vi "Server.vi"() -> ()   [LabVIEW 2020]
uses:
  source/PV Data/NT Scalar (Numeric)/NT Scalar (Numeric).lvclass
  C:/Users/eyw68381/source/repos/pvaccess-labview/labview/source/PV Data/NT Scalar/NT Scalar.lvclass
  C:/Users/eyw68381/source/repos/pvaccess-labview/labview/source/PV Data/NT Base/NT Base.lvclass
  C:/Users/eyw68381/source/repos/pvaccess-labview/labview/source/PV Data/Base/Base.lvclass
  C:/Users/eyw68381/source/repos/pvaccess-labview/labview/source/PV Data/Has Alarm Limits/Has Alarm Limits.lvclass
  C:/Users/eyw68381/source/repos/pvaccess-labview/labview/source/PV Data/Base Interface/Base Interface.lvclass
  C:/Users/eyw68381/source/repos/pvaccess-labview/labview/source/PV Data/Has Control Limits/Has Control Limits.lvclass
  C:/Users/eyw68381/source/repos/pvaccess-labview/labview/source/PV Data/Is Stringifiable/Is Stringifiable.lvclass
  C:/Users/eyw68381/source/repos/pvaccess-labview/labview/source/PV Data/Is Probeable/Is Probeable.lvclass
  C:/Users/eyw68381/source/repos/pvaccess-labview/labview/source/PV Data/Has Alarm/Has Alarm.lvclass
  C:/Users/eyw68381/source/repos/pvaccess-labview/labview/source/PV Data/Has Time Stamp/Has Time Stamp.lvclass
  C:/Users/eyw68381/source/repos/pvaccess-labview/labview/source/PV Data/NT Scalar (Numeric)/NT Scalar (Numeric).lvclass
  source/Server/Server/Server.lvclass
  source/PV Data/Value Fields.ctl
  source/PV Data/PV Data.lvlib
  source/PV Data/Alarm Severity.ctl
  source/PV Data/Display Form.ctl
  source/Server/Server/Post - DBL.vi
  source/Server/Server/Fetch - DBL.vi
  source/Server/Server/Add PV - Any Class.vi
  source/PV Data/NT Scalar (Numeric)/Create - DBL.vi
panel:
  in  "PV name":string="DEV:FLOAT64"
  out "timestamp":timestamp
  in  "Value":dbl min=0.0 max=10.0 step=0.5 format="%.3f"
  in  "Increment":bool
  in  "stop":bool
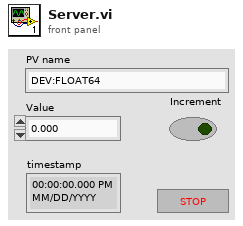
[diagram p1: front panel]
types:
  T1 = typedef "PV Access.lvlib/PV Data.lvlib/Value Fields.ctl" = cluster{"Display":bool, "Control":bool, "Alarm Limits":bool}
  T2 = typedef "PV Access.lvlib/PV Data.lvlib/Alarm Severity.ctl" = enum32{"no", "minor", "major", "record", "invalid", "undefined"}
  T3 = typedef "PV Access.lvlib/PV Data.lvlib/Display Form.ctl" = enum16{"Default", "String", "Binary", "Decimal", "Hex", "Exponential", "Engineering"}
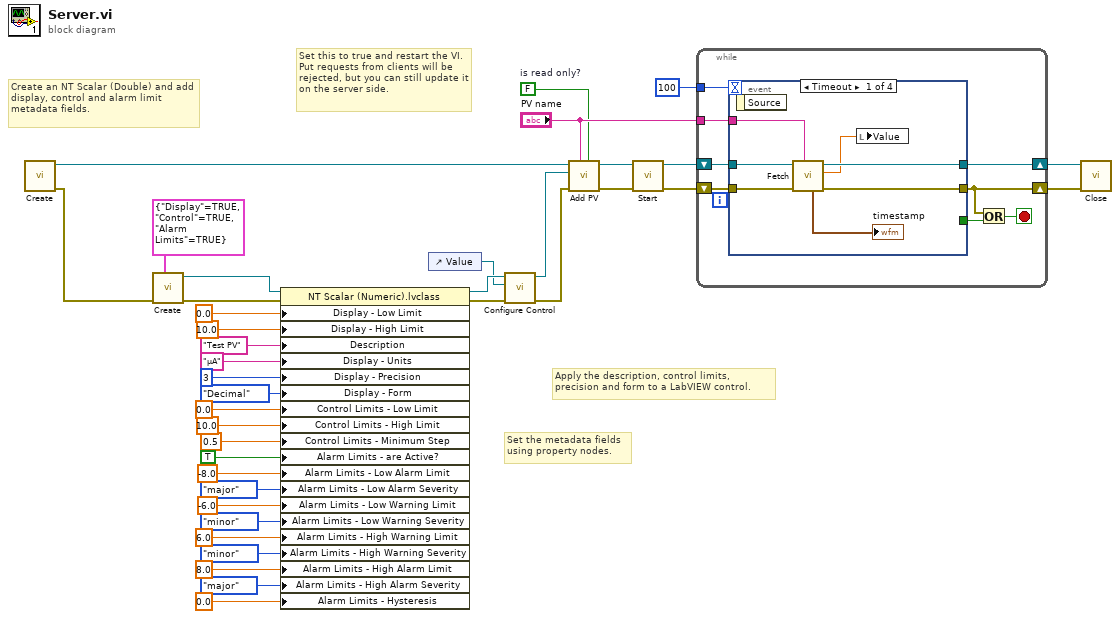
[diagram p0: block diagram]
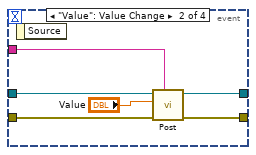
[diagram p2: hidden frame]
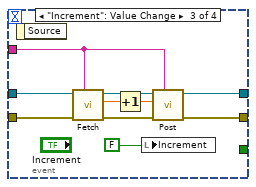
[diagram p3: hidden frame]
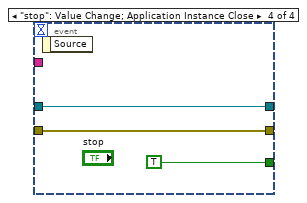
[diagram p4: hidden frame]
diagram:
  w1 = FALSE  # is read only?
  # "Set this to true and restart the VI. Put requests from clients will be rejected, but you can still update it on the server side."
  # "Apply the description, control limits, precision and form to a LabVIEW control."
  # "Set the metadata fields using property nodes."
  # "Create an NT Scalar (Double) and add display, control and alarm limit metadata fields."
  n1 = call "Create.vi"() -> ("error out"=w11:errorcluster, "Server out"=w9:refnum<class "Server.lvclass">)  [unwired: 10 in]
  n2 = call-poly "Create.vi"("fields"=T1 {"Display"=TRUE, "Control"=TRUE, "Alarm Limits"=TRUE}, "error in (no error)"=w11) -> ("error out"=w13:errorcluster, "NT Scalar (Numeric) out"=w12:refnum<class "NT Scalar (Numeric).lvclass">)  [unwired: 8 in]
  n3 = property class="NT Scalar (Numeric).lvclass"(reference=w12, error in=w13, "Display - Low Limit"=0.0 ("Limit Low"), "Display - High Limit"=10.0 ("Limit High"), "Description"="Test PV", "Display - Units"="µA" ("Units"), "Display - Precision"=3 ("Precision"), "Display - Form"=Display_Form."Decimal" ("Form"), "Control Limits - Low Limit"=0.0 ("Limit Low"), "Control Limits - High Limit"=10.0 ("Limit High"), "Control Limits - Minimum Step"=0.5 ("Min Step"), "Alarm Limits - are Active?"=TRUE ("Active"), "Alarm Limits - Low Alarm Limit"=-8.0 ("Low Alarm Limit"), "Alarm Limits - Low Alarm Severity"=Alarm_Severity."major" ("Severity"), "Alarm Limits - Low Warning Limit"=-6.0 ("Low Warning Limit"), "Alarm Limits - Low Warning Severity"=Alarm_Severity."minor" ("Severity"), "Alarm Limits - High Warning Limit"=6.0 ("High Warning Limit"), "Alarm Limits - High Warning Severity "=Alarm_Severity."minor" ("Severity"), "Alarm Limits - High Alarm Limit"=8.0 ("High Alarm Limit"), "Alarm Limits - High Alarm Severity"=Alarm_Severity."major" ("Severity"), "Alarm Limits - Hysteresis"=0.0 ("Hysteresis")) -> (reference out=w25:refnum<class "NT Scalar (Numeric).lvclass">, error out=w26:errorcluster)
  n4 = control-ref of="Value"() -> (w14:refnum<vi>)
  n5 = call-dynamic "Configure Control.vi"("error in (no error)"=w26, "control"=w14, "NT Scalar (Numeric) in"=w25) -> ("error out"=w7:errorcluster, "NT Scalar (Numeric) out"=w6:refnum<class "NT Scalar (Numeric).lvclass">)  [unwired: 6 in, 1 out]
  n6 = call-poly "Add PV.vi"("is read only? (F)"=w1, "PV name"="PV name", "error in (no error)"=w7, "initial value"=w6, "Server in"=w9) -> ("error out"=w5:errorcluster, "Server out"=w4:refnum<class "Server.lvclass">)  [unwired: 4 in, 1 out]
  n7 = call-dynamic "Start.vi"("error in (no error)"=w5, "Server in"=w4) -> ("error out"=w2:errorcluster, "Server out"=w3:refnum<class "Server.lvclass">)  [unwired: 8 in]
  n8 = while {
    tunnel: "PV name" -> [w45]
    shift-right: [w43] -> w36
    shift-left: w3 -> [w44]
    shift-right: [w40] -> w37
    shift-left: w2 -> [w46]
    tunnel: 100 ("Numeric") -> [w39]
    stop <- w41 stop-if-true
    n9 = event shown="[0] Timeout" {
      selector: _ -> [_ _ _ _]
      dyn-events: _ -> [_ _ _ _]
      timeout: w39 -> [_ _ _ _]
      tunnel: w46 -> [w53 w59 w69 w71]
      tunnel: w45 -> [w48 w58 w62 _]
      tunnel: w44 -> [w52 w57 w68 w70]
      tunnel: [w50 w55 w60 w71] -> w40
      tunnel: [w51 w56 w61 w70] -> w43
      tunnel: [_ _ _ TRUE] -> w42
      event Timeout {
        n10 = event-data() -> ()  [unwired: 1 in, 1 out]
        n11 = call-poly "Fetch.vi"("PV name"=w48, "error in"=w53, "Server in"=w52) -> ("error out"=w50:errorcluster, "value"=w49:dbl, "Server out"=w51:refnum<class "Server.lvclass">, "timestamp"=→"timestamp":timestamp)  [unwired: 4 in, 1 out]
        n12 = local write "Value"(w49) -> ()
      }
      event "Value": Value Change {
        n13 = event-data() -> ()  [unwired: 1 in, 1 out]
        n14 = call-poly "Post.vi"("PV name"=w58, "error in (no error)"=w59, "value"="Value", "Server in"=w57) -> ("error out"=w55:errorcluster, "Server out"=w56:refnum<class "Server.lvclass">)  [unwired: 6 in]
      }
      event "Increment": Value Change {
        n15 = event-data() -> ()  [unwired: 1 in, 1 out]
        n16 = call-poly "Fetch.vi"("PV name"=w62, "error in"=w69, "Server in"=w68) -> ("error out"=w65:errorcluster, "value"=w66:dbl, "Server out"=w63:refnum<class "Server.lvclass">)  [unwired: 4 in, 2 out]
        n17 = Increment(x=w66) -> (x+1=w64:dbl)
        n18 = local write "Increment"(FALSE ("Increment")) -> ()
        n19 = call-poly "Post.vi"("PV name"=w62, "error in (no error)"=w65, "value"=w64, "Server in"=w63) -> ("error out"=w60:errorcluster, "Server out"=w61:refnum<class "Server.lvclass">)  [unwired: 6 in]
      }
      event "stop": Value Change; Application Instance Close {
        n20 = event-data() -> ()  [unwired: 1 in, 1 out]
      }
    }
    n21 = Or(x=w40, y=w42) -> (x .or. y?=w41:bool)
  }
  n22 = call-dynamic "Close.vi"("error in"=w37, "Server in"=w36) -> ()  [unwired: 9 in, 1 out]
